vi "SLSC Parse Capabilities File.vi"(8 "error in":errorcluster, 11 "module capabilities JSON string":string) -> (0 "error out":errorcluster, 2 "Raw Partition?":bool, 3 "SLSC EDS module":T1)   [LabVIEW 2020]
doc: "This SLSC capabilities string parser deserializes a module's JSON capabilities string as read using SLSC Read NVMEM.vi example (*.bin)) and converts it to a cluster."
uses:
  EDSjsonStructure.ctl
  enum.ctl
  property.ctl
  command.ctl
  scale.ctl
  physicalChannel.ctl
  register.ctl
  <vilib>/addons/_JKI.lib/Serialization/JSON/JKI JSON Serialization.lvlib
panel:
  out "First Region":string
  out "result string":string
  # "not working\nregisterMap->registers->initialValue"
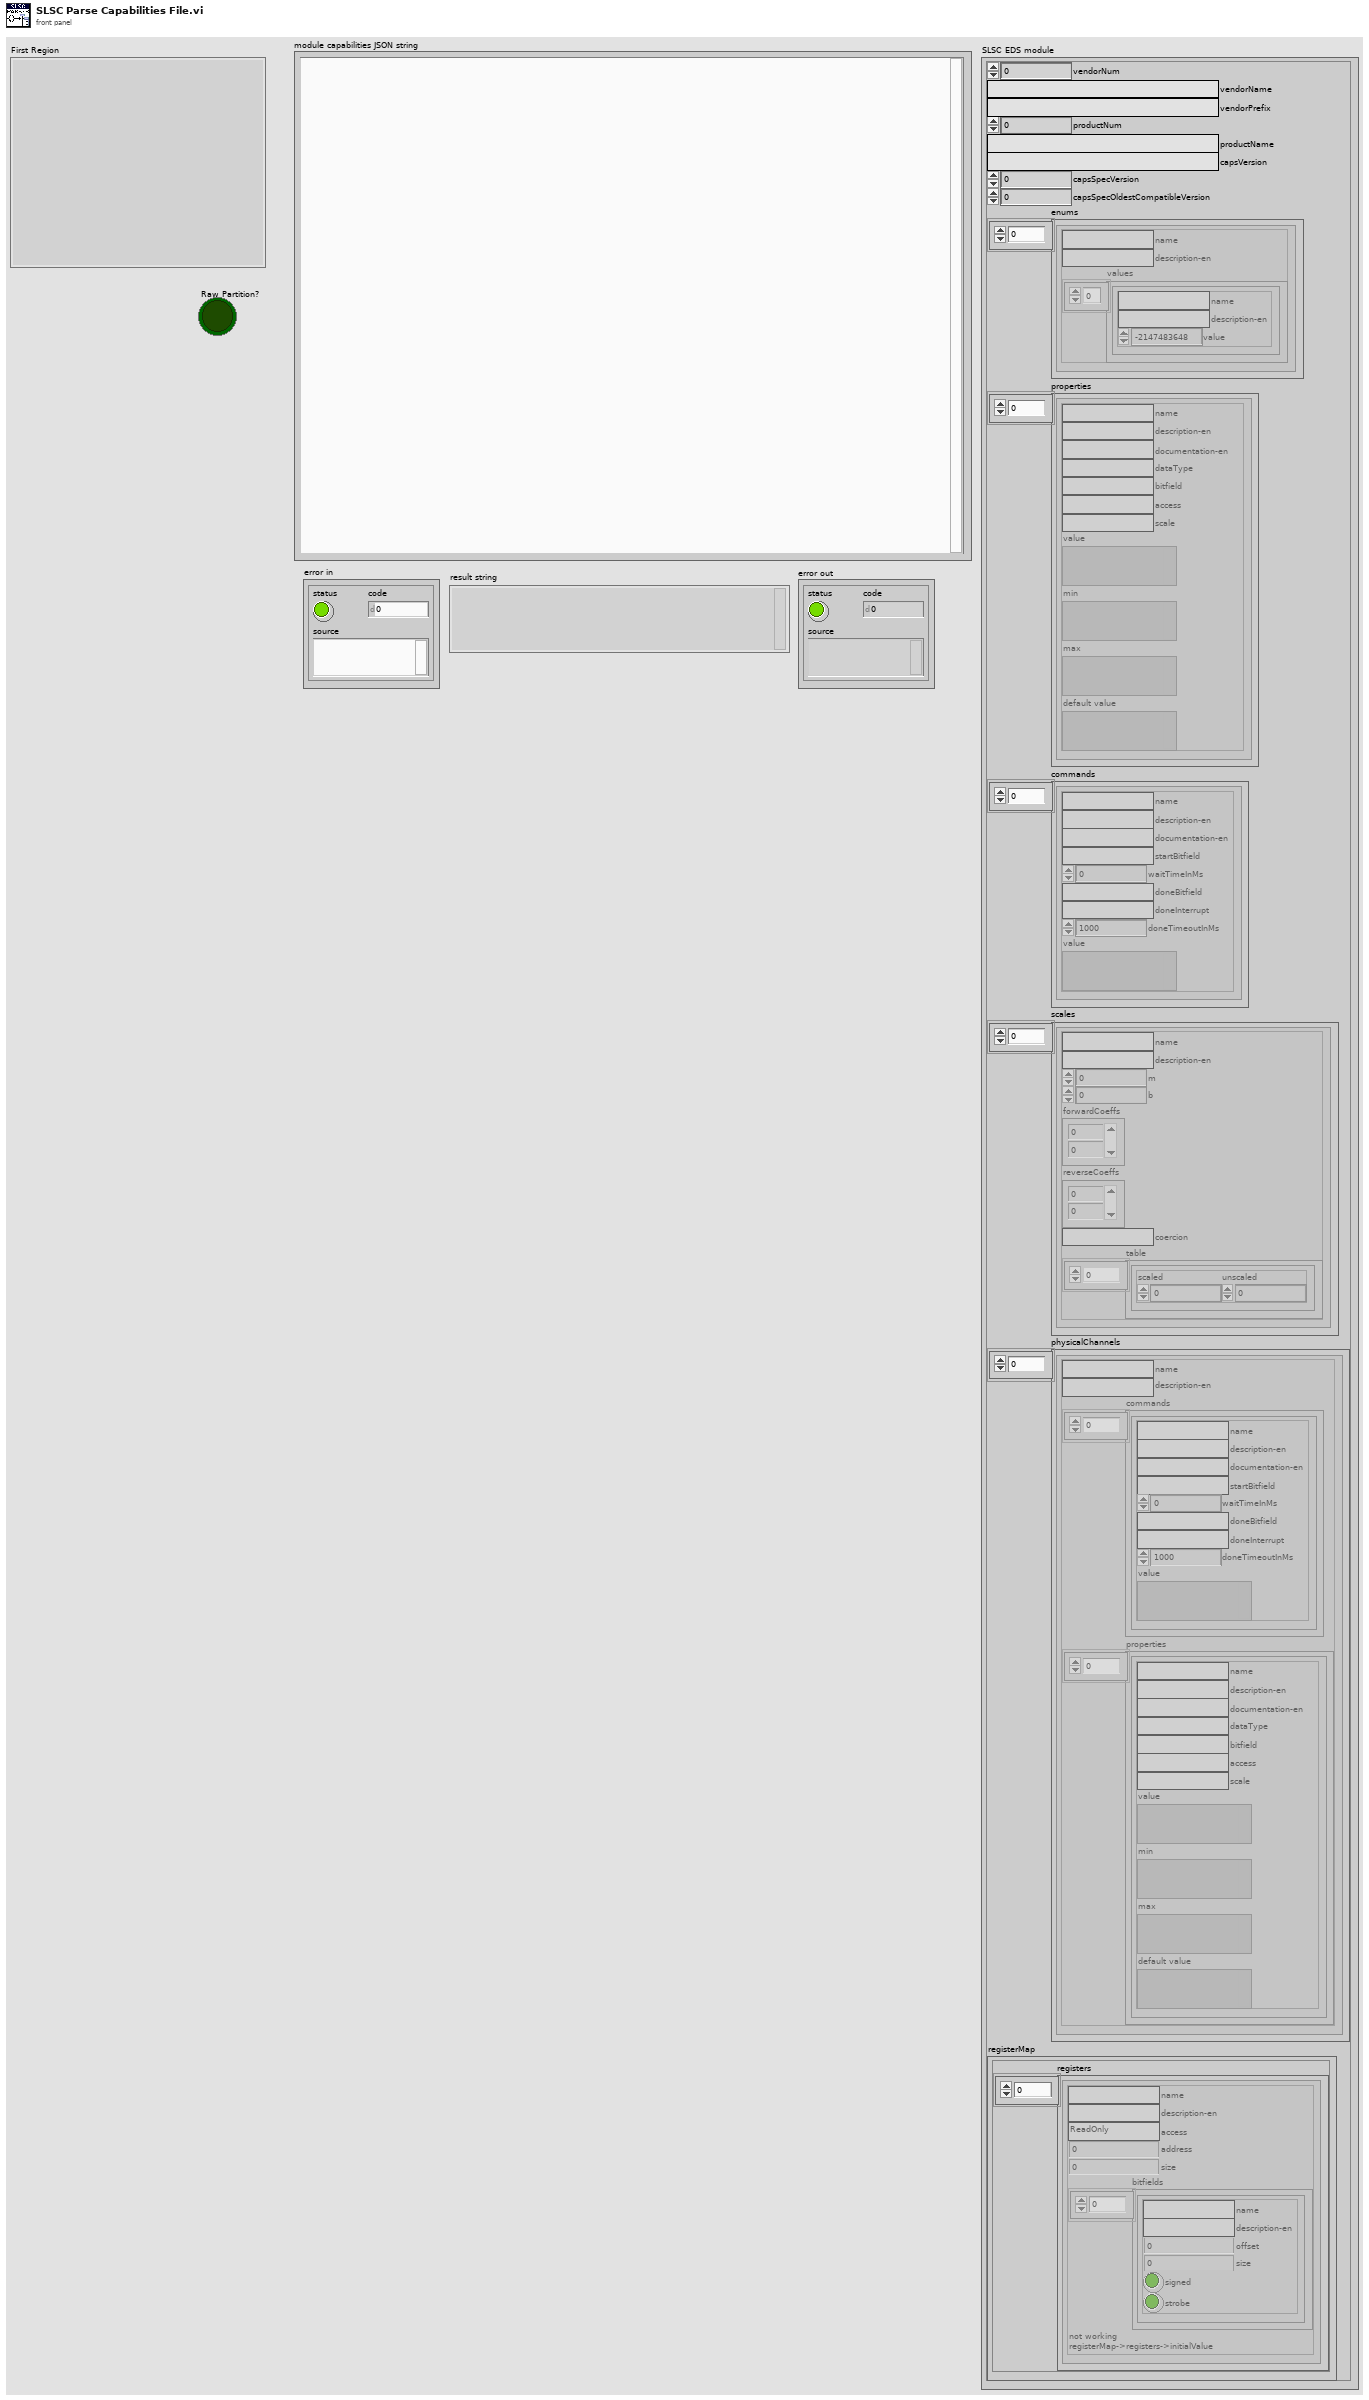
[diagram p1: front panel]
types:
  T1 = typedef "EDSjsonStructure.ctl" = cluster{"vendorNum":u32, "vendorName":string, "vendorPrefix":string, "productNum":u32, "productName":string, "capsVersion":string, "capsSpecVersion":u32, "capsSpecOldestCompatibleVersion":u32, "enums":T2[], "properties":T3[], "commands":T4[], "scales":T5[], "physicalChannels":T6[], "registerMap":cluster{"registers":T7[]}}
  T2 = typedef "enum.ctl" = cluster{"name":string, "description-en":string, "values":cluster{"name":string, "description-en":string, "value":i32}[]}
  T3 = typedef "property.ctl" = cluster{"name":string, "description-en":string, "documentation-en":string, "dataType":string, "bitfield":string, "access":string, "scale":string, "value":variant, "min":variant, "max":variant, "default value":variant}
  T4 = typedef "command.ctl" = cluster{"name":string, "description-en":string, "documentation-en":string, "startBitfield":string, "waitTimeInMs":i32, "doneBitfield":string, "doneInterrupt":string, "doneTimeoutInMs":i32, "value":variant}
  T5 = typedef "scale.ctl" = cluster{"name":string, "description-en":string, "m":dbl, "b":dbl, "forwardCoeffs":dbl[], "reverseCoeffs":dbl[], "coercion":string, "table":cluster{"scaled":dbl, "unscaled":dbl}[]}
  T6 = typedef "physicalChannel.ctl" = cluster{"name":string, "description-en":string, "commands":T4[], "properties":T3[]}
  T7 = typedef "register.ctl" = cluster{"name":string, "description-en":string, "access":string, "address":u32, "size":u32, "bitfields":cluster{"name":string, "description-en":string, "offset":u32, "size":u32, "signed":bool, "strobe":bool}[]}
  T8 = cluster{"areas":cluster{"name":string, "offsets":i32[], "size":i32}[]}
  T9 = cluster{"name":string, "offsets":i32[], "size":i32}[]
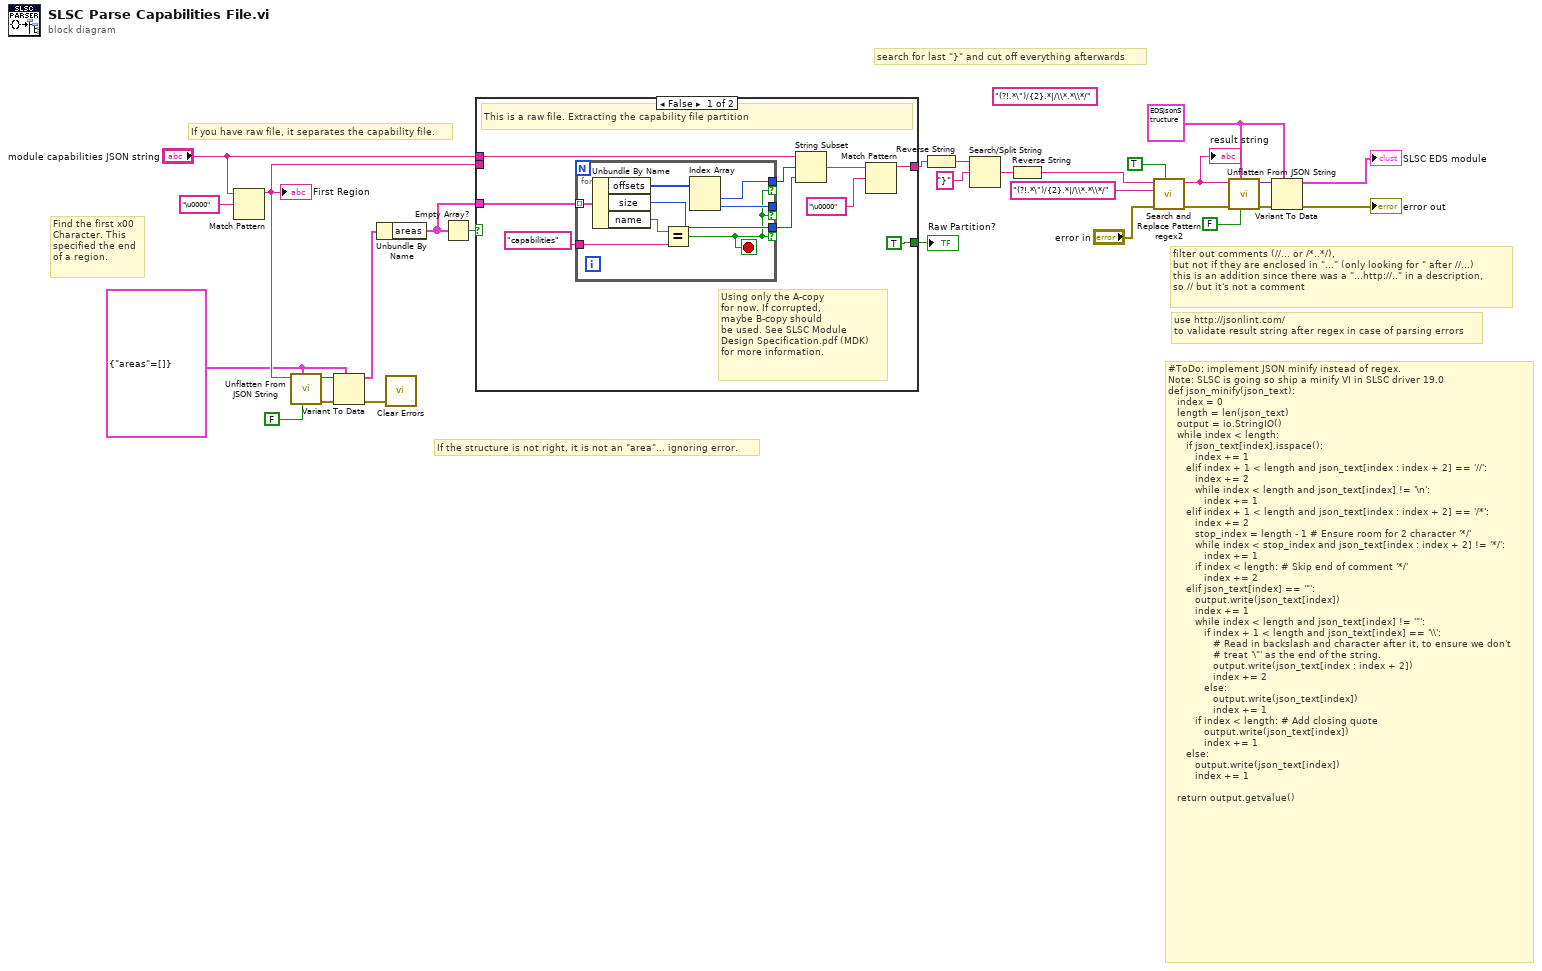
[diagram p0: block diagram]
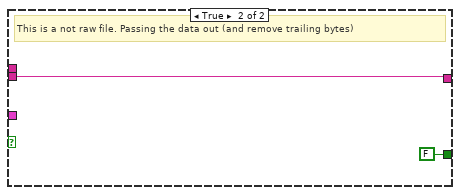
[diagram p2: hidden frame]
diagram:
  (unwired) "(?!.*\")/{2}.*|/\\*.*\\*/" ("regular expression (\"\")")
  w16 = T1 {"vendorNum"=0, "vendorName"="", "vendorPrefix"="", "productNum"=0, "productName"="", "capsVersion"="", "capsSpecVersion"=0, "capsSpecOldestCompatibleVersion"=0, "enums"=[], "properties"=[], "commands"=[], "scales"=[], "physicalChannels"=[], "registerMap"={"registers"=[]}} ("ESDmoduleOptElements")
  w6 = T8 {"areas"=[]}
  # "If the structure is not right, it is not an \"area\"... ignoring error."
  # "If you have raw file, it separates the capability file."
  # "search for last \"}\" and cut off everything afterwards"
  # "use http://jsonlint.com/\nto validate result string after regex in case of parsing errors"
  # "filter out comments (//... or /*..*/),\nbut not if they are enclosed in \"...\" (only looking for \" after //...)\nthis is an addition since there was a \"...http://..\" in a description, \nso // but it's not a comment"
  # "Find the first x00 \nCharacter. This \nspecified the end\nof a region."
  # "#ToDo: implement JSON minify instead of regex.\nNote: SLSC is going so ship a minify VI in SLSC driver 19.0\ndef json_minify(json_text):\n   index = 0\n   length = len(json_text)\n   output = io.StringIO()\n   while index < length:\n      if json_text[index].isspace():\n         index += 1\n      elif index + 1 < length and json_text[index : index + 2] == '//':\n         index += 2\n         while index < length and json_text[index] != '\\n':\n            index += 1\n      elif index + 1 < length and json_text[index : index + 2] == '/*':\n         index += 2\n         stop_index = length - 1 # Ensure room for 2 character '*/'\n         while index < stop_index and json_text[index : index + 2] != '*/':\n            index += 1\n         if index < length: # Skip end of comment '*/'\n            index += 2\n      elif json_text[index] == '\"':\n         output.write(json_text[index])\n         index += 1\n         while index < length and json_text[index] != '\"':\n            if index + 1 < length and json_text[index] == '\\\\':\n               # Read in backslash and character after it, to ensure we don't\n               # treat '\\\"' as the end of the string.\n               output.write(json_text[index : index + 2])\n               index += 2\n            else:\n               output.write(json_text[index])\n               index += 1\n         if index < length: # Add closing quote\n            output.write(json_text[index])\n            index += 1\n      else:\n         output.write(json_text[index])\n         index += 1\n\n   return output.getvalue()"
  n1 = Match Pattern(string="module capabilities JSON string", regular expression="\u0000" ("search string")) -> (before substring=w7:string)  [unwired: 1 in, 3 out]
  "First Region" <- w7
  n2 = call <vilib>:"Unflatten From JSON String.vi"("Nulls as Defaults (F)"=FALSE, "Type and Defaults"=w6, "JSON String"=w7) -> ("error out"=w8:errorcluster, "Variant"=w4:variant)  [unwired: 7 in]
  n3 = Variant To Data(error in=w8, type=w6, Variant=w4) -> (data=w3:T8, error out=w2:errorcluster)
  n4 = Unbundle By Name(w3) -> ("areas"=w26:T9)
  n5 = call <vilib>:"Clear Errors.vi"("error in (no error)"=w2) -> ()  [unwired: 5 in, 2 out]
  n6 = Empty Array?(array=w26) -> (empty?=w23:bool)
  n7 = case shown="False" w23 {
    tunnel: w26 -> [w37 _]
    tunnel: "module capabilities JSON string" -> [w35 _]
    tunnel: [w30 w47] -> w9
    tunnel: w7 -> [_ w47]
    tunnel: [TRUE ("raw?") FALSE ("raw?")] -> w10
    frame False {
      # "Using only the A-copy\nfor now. If corrupted,\nmaybe B-copy should \nbe used. See SLSC Module\nDesign Specification.pdf (MDK)\nfor more information."
      # "This is a raw file. Extracting the capability file partition"
      n8 = for {
        tunnel: w37 -> [w45] mode=indexing
        tunnel: "capabilities" ("y") -> [w42]
        tunnel: [w41] -> w33 if=w38
        tunnel: [w40] -> w34 if=w38
        tunnel: [w39] -> _ if=w38
        stop <- w38 stop-if-true
        n9 = Unbundle By Name(w45) -> ("offsets"=w43:i32[], "size"=w41:i32, "name"=w44:string)
        n10 = Equal?(x=w44, y=w42) -> (x = y?=w38:bool)
        n11 = Index Array(array=w43) -> (element #1=w40:i32, element #2=w39:i32)  [unwired: 2 in]
      }
      n12 = String Subset(string=w35, offset (0)=w34, length (rest)=w33) -> (substring=w31:string)
      n13 = Match Pattern(string=w31, regular expression="\u0000" ("search string")) -> (before substring=w30:string)  [unwired: 1 in, 3 out]
    }
    frame True {
      # "This is a not raw file. Passing the data out (and remove trailing bytes)"
    }
  }
  "Raw Partition?" <- w10
  n14 = Reverse String(1:w9) -> (0:w14:string)
  n15 = Search/Split String(string=w14, search string/char (-)="}") -> (match + rest of string=w11:string)  [unwired: 1 in, 2 out]
  n16 = Reverse String(1:w11) -> (0:w12:string)
  n17 = call "Search and Replace Pattern regex2.vi"("replace all? (F)"=TRUE, "error in"="error in", "regular expression (\"\")"="(?!.*\")/{2}.*|/\\*.*\\*/" ("regular expression (\"\")"), "string"=w12) -> ("error out"=w15:errorcluster, "result string"=w20:string)  [unwired: 5 in, 1 out]
  "result string" <- w20
  n18 = call <vilib>:"Unflatten From JSON String.vi"("Nulls as Defaults (F)"=FALSE, "Type and Defaults"=w16, "error in (no error)"=w15, "JSON String"=w20) -> ("error out"=w19:errorcluster, "Variant"=w18:variant)  [unwired: 6 in]
  n19 = Variant To Data(error in=w19, type=w16, Variant=w18) -> (data=→"SLSC EDS module":T1, error out=→"error out":errorcluster)
